vi "Add Configuration Controls.vi"(0 "New Code Module":path, 1 "vi reference":refnum<vi>, 2 "Configuration Ctl Refnum":refnum<vi>, 11 "error in (no error)":errorcluster) -> (4 "Controls Reference":refnum<vi>[](array[refnum]), 15 "error out":errorcluster)   [LabVIEW 2021, in "Migrator.lvlib"]
uses:
  Migrator.lvlib
  Migrator Reusables/Migrator Reusables.lvlib
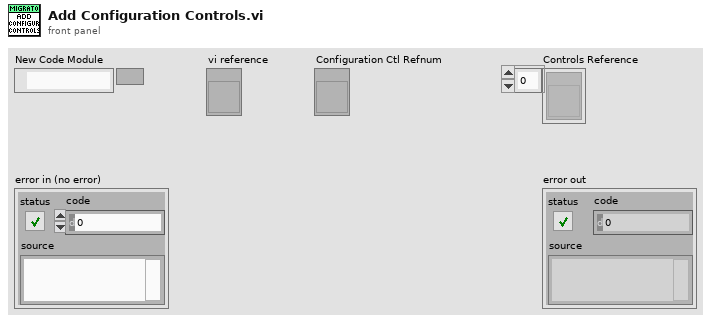
[diagram p1: front panel]
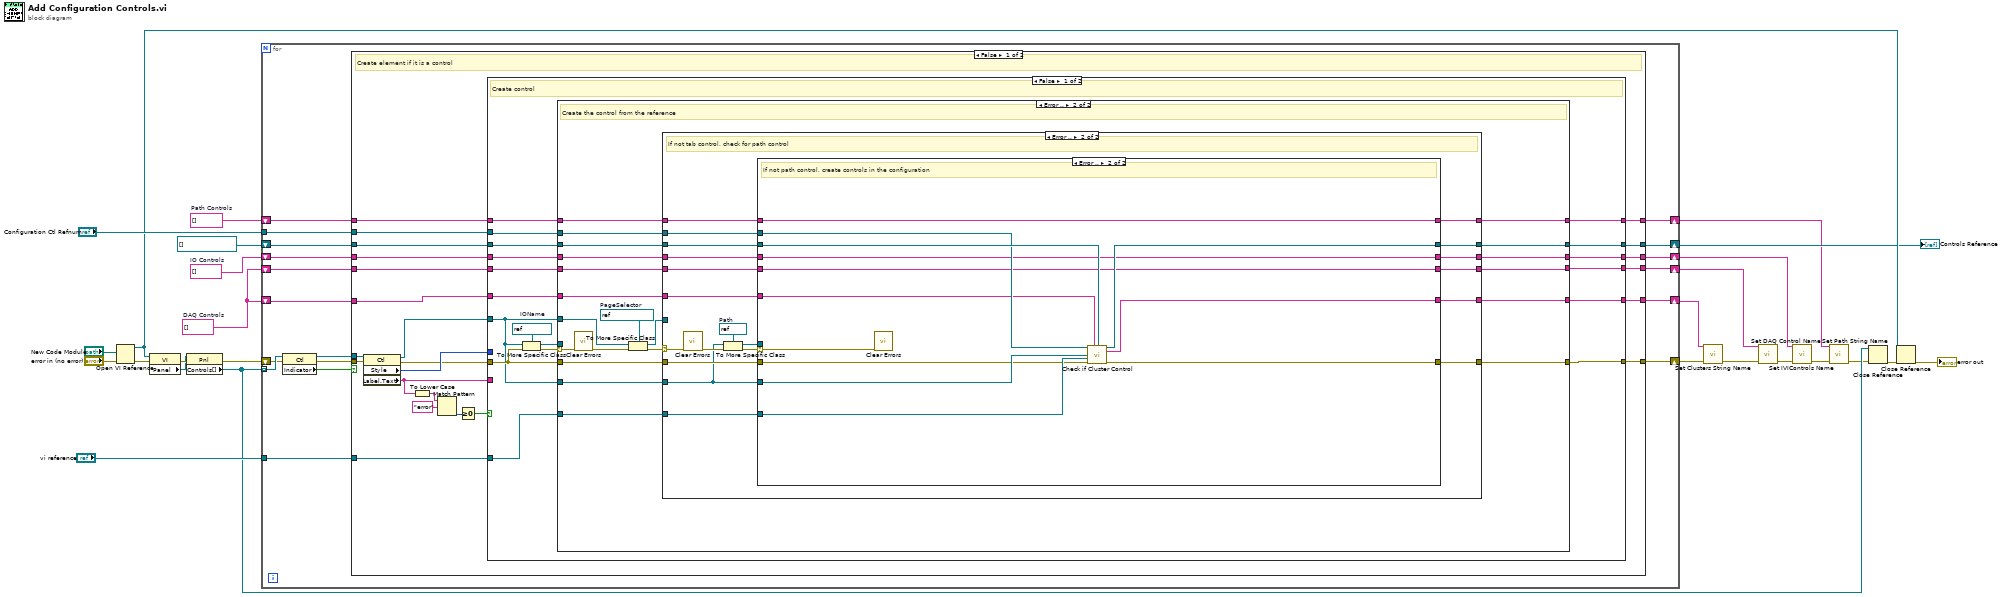
[diagram p0: block diagram]
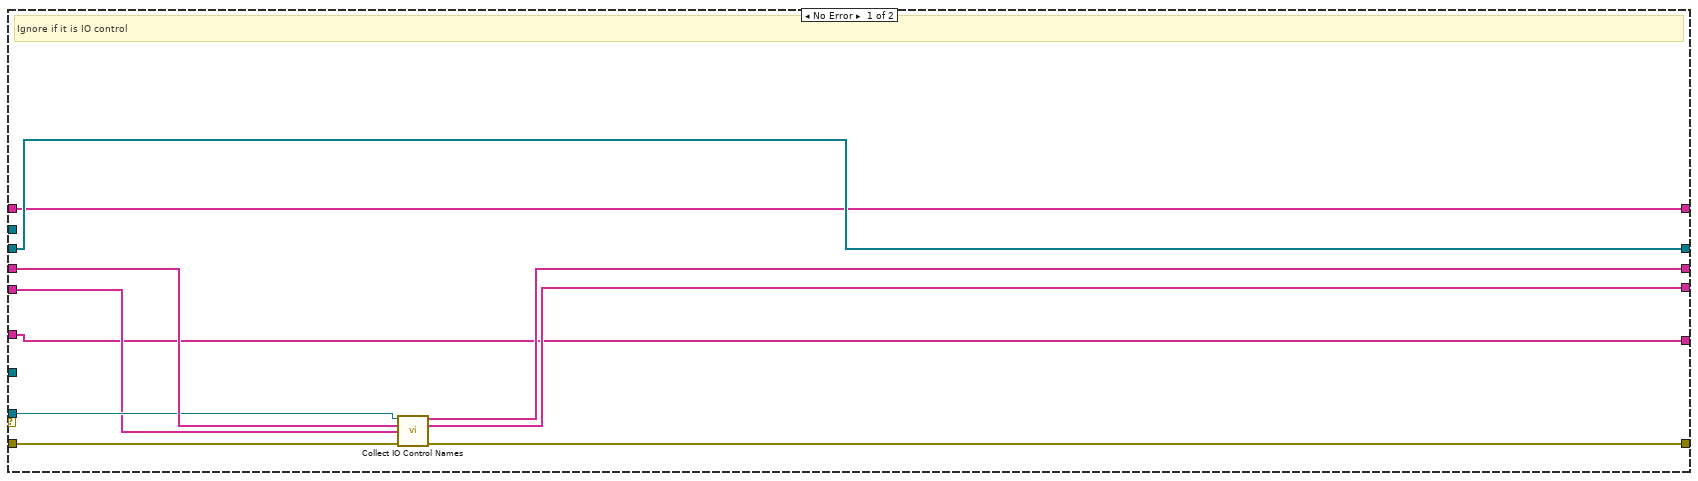
[diagram p2: hidden frame]
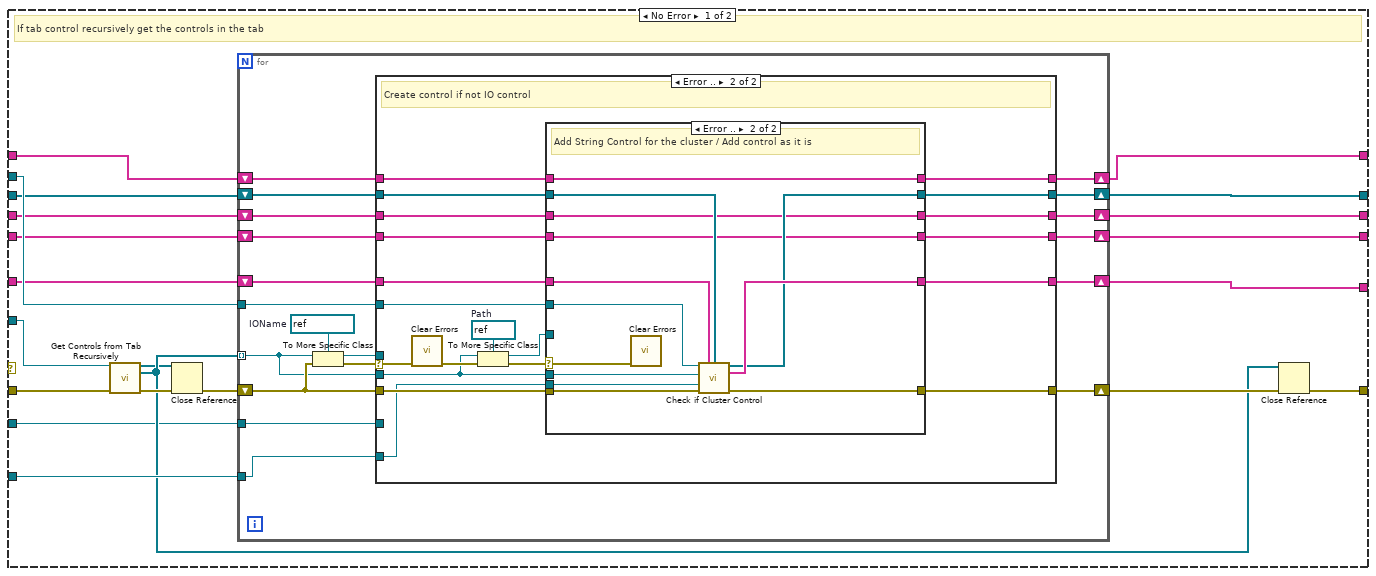
[diagram p3: hidden frame]
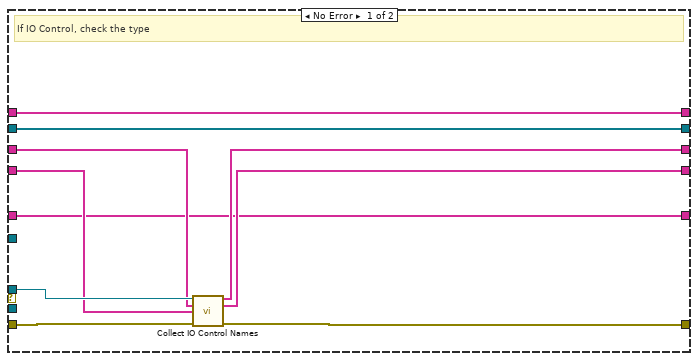
[diagram p4: hidden frame]
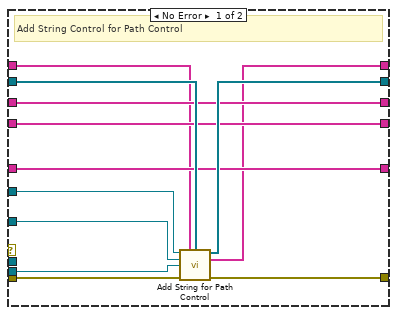
[diagram p5: hidden frame]
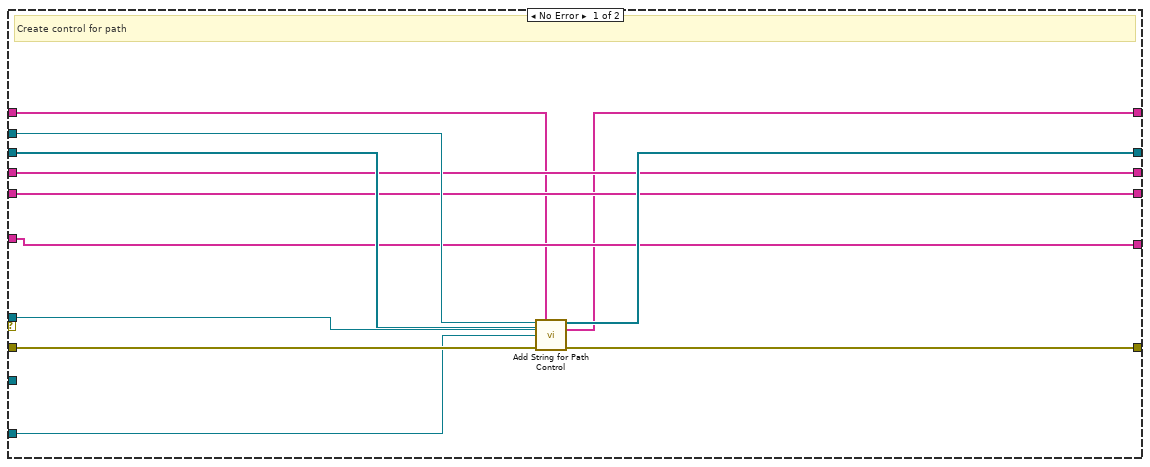
[diagram p6: hidden frame]
diagram:
  w4 = string[] []  # Path Controls
  w8 = string[] []  # DAQ Controls
  w12 = string[] []  # IO Controls
  n1 = Open VI Reference(vi path="New Code Module", error in (no error)="error in (no error)") -> (vi reference=w18:refnum<vi>, error out=w16:errorcluster)  [unwired: 4 in]
  n2 = property class="VI"(reference=w18, error in=w16) -> (error out=w20:errorcluster, "Panel"=w19:refnum<vi>)  [unwired: 1 out]
  n3 = property class="Pnl"(reference=w19, error in=w20) -> (error out=w15:errorcluster, "Controls[]"=w17:refnum<vi>[])  [unwired: 1 out]
  n4 = for {
    tunnel: w17 -> [w42] mode=indexing
    shift-right: [w43] -> w5
    shift-left: w15 -> [w40]
    tunnel: "Configuration Ctl Refnum" -> [w44]
    tunnel: "vi reference" -> [w37]
    shift-right: [w36] -> w14
    shift-left: refnum<vi>[] [] -> [w35]
    shift-right: [w33] -> w13
    shift-left: w12 -> [w34]
    shift-right: [w31] -> w10
    shift-left: w8 -> [w32]
    shift-right: [w30] -> w7
    shift-left: w8 -> [w29]
    shift-right: [w27] -> w3
    shift-left: w4 -> [w28]
    n5 = property class="Ctl"(reference=w42, error in=w40) -> (reference out=w38:refnum<vi>, error out=w39:errorcluster, "Indicator"=w41:bool)
    n6 = case shown="False" w41 {
      tunnel: w44 -> [w66 _]
      tunnel: w39 -> [w65 w268]
      tunnel: w38 -> [w63 _]
      tunnel: [w62 w268] -> w43
      tunnel: w37 -> [w55 _]
      tunnel: [w54 w267] -> w36
      tunnel: w35 -> [w53 w267]
      tunnel: w34 -> [w52 w266]
      tunnel: [w51 w266] -> w33
      tunnel: w32 -> [w50 w265]
      tunnel: [w49 w265] -> w31
      tunnel: [w48 w264] -> w30
      tunnel: w29 -> [w47 w264]
      tunnel: w28 -> [w46 w263]
      tunnel: [w45 w263] -> w27
      frame False {
        # "Create element if it is a control"
        n7 = property class="Ctl"(reference=w63, error in=w65) -> (reference out=w56:refnum<vi>, error out=w64:errorcluster, "Style"=w67:u32, "Label.Text"=w61:string)
        n8 = To Lower Case(string=w61) -> (all lower case string=w57:string)
        n9 = Match Pattern(string=w57, regular expression="error") -> (offset past match=w59:i32)  [unwired: 1 in, 3 out]
        n10 = Greater Or Equal To 0?(x=w59) -> (x >= 0?=w58:bool)
        n11 = case shown="False" w58 {
          tunnel: w67 -> [_ _]
          tunnel: w66 -> [w83 _]
          tunnel: w64 -> [w85 w262]
          tunnel: w56 -> [w78 _]
          tunnel: w61 -> [_ _]
          tunnel: [w84 w262] -> w62
          tunnel: w55 -> [w82 _]
          tunnel: [w77 w261] -> w54
          tunnel: w53 -> [w76 w261]
          tunnel: w52 -> [w75 w260]
          tunnel: [w74 w260] -> w51
          tunnel: w50 -> [w73 w259]
          tunnel: [w72 w259] -> w49
          tunnel: [w71 w258] -> w48
          tunnel: w47 -> [w70 w258]
          tunnel: w46 -> [w69 w257]
          tunnel: [w68 w257] -> w45
          frame False {
            w81 = refnum<vi> refnum  # IOName
            # "Create control"
            n12 = To More Specific Class(target class=w81, reference=w78, error in=w85) -> (specific class reference=w79:refnum<vi>, error out=w80:errorcluster)
            n13 = case shown="Error .." w80 {
              selector: w80 -> [_ w113]
              tunnel: w82 -> [_ w110]
              tunnel: w78 -> [_ w116]
              tunnel: w83 -> [_ w115]
              tunnel: [w95 w114] -> w84
              tunnel: w85 -> [w91 w112]
              tunnel: w79 -> [w90 _]
              tunnel: w78 -> [_ w108]
              tunnel: [w94 w105] -> w77
              tunnel: w76 -> [w94 w104]
              tunnel: w75 -> [w93 w103]
              tunnel: [w92 w102] -> w74
              tunnel: w73 -> [w89 w101]
              tunnel: [w88 w100] -> w72
              tunnel: [w87 w99] -> w71
              tunnel: w70 -> [w87 w98]
              tunnel: w69 -> [w86 w97]
              tunnel: [w86 w96] -> w68
              frame No Error {
                # "Ignore if it is IO control"
                n14 = call "Collect IO Control Names.vi"("IO Control"=w90, "IO Controls in"=w93, "DAQ Controls in"=w89, "error in (no error)"=w91) -> ("IO Controls out"=w92:string[], "DAQ Controls out"=w88:string[], "error out"=w95:errorcluster)  [unwired: 9 in]
              }
              frame Error {
                w111 = refnum<vi> refnum  # PageSelector
                # "Create the control from the reference"
                n15 = call <vilib>:"Clear Errors.vi"("error in (no error)"=w113) -> ("error out"=w109:errorcluster)  [unwired: 5 in, 1 out]
                n16 = To More Specific Class(target class=w111, reference=w108, error in=w109) -> (specific class reference=w106:refnum<vi>, error out=w107:errorcluster)
                n17 = case shown="Error .." w107 {
                  selector: w107 -> [_ w223]
                  tunnel: w110 -> [w134 w229]
                  tunnel: w116 -> [w123 w214]
                  tunnel: w115 -> [w133 w227]
                  tunnel: [w137 w228] -> w114
                  tunnel: w112 -> [w136 w224]
                  tunnel: w106 -> [w135 _]
                  tunnel: [w121 w230] -> w105
                  tunnel: w104 -> [w122 w231]
                  tunnel: w103 -> [w132 w219]
                  tunnel: [w131 w216] -> w102
                  tunnel: w101 -> [w125 w218]
                  tunnel: [w124 w215] -> w100
                  tunnel: [w119 w226] -> w99
                  tunnel: w98 -> [w120 w225]
                  tunnel: w97 -> [w118 w213]
                  tunnel: [w117 w212] -> w96
                  frame No Error {
                    # "If tab control recursively get the controls in the tab"
                    n18 = call "Get Controls from Tab Recursively.vi"("PageSel Refnum"=w135, "error in (no error)"=w136) -> ("Indicators in Tab"=w126:refnum<vi>[], "Controls in Tab"=w127:refnum<vi>[], "error out"=w129:errorcluster)  [unwired: 11 in]
                    n19 = Close Reference(reference=w126, error in (no error)=w129) -> (error out=w128:errorcluster)
                    n20 = for {
                      tunnel: w127 -> [w142] mode=indexing
                      tunnel: w134 -> [w145]
                      tunnel: w133 -> [w147]
                      shift-right: [w150] -> w131
                      shift-left: w132 -> [w154]
                      shift-right: [w151] -> w130
                      shift-left: w128 -> [w148]
                      shift-right: [w149] -> w124
                      shift-left: w125 -> [w152]
                      tunnel: w123 -> [w146]
                      shift-right: [w143] -> w121
                      shift-left: w122 -> [w144]
                      shift-right: [w140] -> w119
                      shift-left: w120 -> [w141]
                      shift-right: [w138] -> w117
                      shift-left: w118 -> [w139]
                      w156 = refnum<vi> refnum  # IOName
                      n21 = To More Specific Class(target class=w156, reference=w142, error in=w148) -> (specific class reference=w155:refnum<vi>, error out=w153:errorcluster)
                      n22 = case shown="Error .." w153 {
                        selector: w153 -> [_ w176]
                        tunnel: w155 -> [w166 _]
                        tunnel: w154 -> [w165 w172]
                        tunnel: w152 -> [w164 w170]
                        tunnel: [w163 w182] -> w151
                        tunnel: [w162 w171] -> w150
                        tunnel: [w161 w169] -> w149
                        tunnel: w148 -> [w160 w183]
                        tunnel: w147 -> [_ w184]
                        tunnel: w146 -> [_ _]
                        tunnel: w145 -> [_ w181]
                        tunnel: [w159 w179] -> w143
                        tunnel: w144 -> [w159 w180]
                        tunnel: w142 -> [_ w174]
                        tunnel: w141 -> [w158 w186]
                        tunnel: [w158 w185] -> w140
                        tunnel: w139 -> [w157 w168]
                        tunnel: [w157 w167] -> w138
                        frame No Error {
                          # "If IO Control, check the type"
                          n23 = call "Collect IO Control Names.vi"("IO Control"=w166, "IO Controls in"=w165, "DAQ Controls in"=w164, "error in (no error)"=w160) -> ("IO Controls out"=w162:string[], "DAQ Controls out"=w161:string[], "error out"=w163:errorcluster)  [unwired: 9 in]
                        }
                        frame Error {
                          w178 = refnum<vi> refnum  # Path
                          # "Create control if not IO control"
                          n24 = call <vilib>:"Clear Errors.vi"("error in (no error)"=w176) -> ("error out"=w175:errorcluster)  [unwired: 5 in, 1 out]
                          n25 = To More Specific Class(target class=w178, reference=w174, error in=w175) -> (specific class reference=w173:refnum<vi>, error out=w177:errorcluster)
                          n26 = case shown="Error .." w177 {
                            selector: w177 -> [_ w211]
                            tunnel: w186 -> [w189 w210]
                            tunnel: [w189 w209] -> w185
                            tunnel: w184 -> [w195 w208]
                            tunnel: w183 -> [w198 w207]
                            tunnel: [w197 w206] -> w182
                            tunnel: w174 -> [_ w205]
                            tunnel: w181 -> [w194 w204]
                            tunnel: w180 -> [w193 w203]
                            tunnel: [w192 w202] -> w179
                            tunnel: w173 -> [w196 _]
                            tunnel: [w191 w201] -> w171
                            tunnel: w172 -> [w191 w201]
                            tunnel: w170 -> [w190 w200]
                            tunnel: [w190 w200] -> w169
                            tunnel: w168 -> [w188 w199]
                            tunnel: [w187 w199] -> w167
                            frame No Error {
                              # "Add String Control for Path Control"
                              n27 = call "Add String for Path Control.vi"("String Controls in"=w195, "String Names in"=w188, "Controls Ref IN"=w193, "Path Refnum"=w196, "vi reference"=w194, "error in (no error)"=w198) -> ("Controls Ref Out"=w192:refnum<vi>[], "String Names Out"=w187:string[], "error out"=w197:errorcluster)  [unwired: 7 in]
                            }
                            frame Error {
                              # "Add String Control for the cluster / Add control as it is"
                              n28 = call <vilib>:"Clear Errors.vi"("error in (no error)"=w211) -> ()  [unwired: 5 in, 2 out]
                              n29 = call "Check if Cluster Control.vi"(0:"String Controls in"=w208, 1:"String Controls in"=w210, "Controls Ref IN"=w203, "Ctl Refnum"=w205, "vi reference"=w204, "error in"=w207) -> ("Controls Ref Out"=w202:refnum<vi>[], "String Controls out"=w209:string[], "error out"=w206:errorcluster)  [unwired: 7 in]
                            }
                          }
                        }
                      }
                    }
                    n30 = Close Reference(reference=w127, error in (no error)=w130) -> (error out=w137:errorcluster)
                  }
                  frame Error {
                    w220 = refnum<vi> refnum  # Path
                    # "If not tab control, check for path control"
                    n31 = call <vilib>:"Clear Errors.vi"("error in (no error)"=w223) -> ("error out"=w222:errorcluster)  [unwired: 5 in, 1 out]
                    n32 = To More Specific Class(target class=w220, reference=w214, error in=w222) -> (specific class reference=w217:refnum<vi>, error out=w221:errorcluster)
                    n33 = case shown="Error .." w221 {
                      selector: w221 -> [_ w247]
                      tunnel: w231 -> [w239 w256]
                      tunnel: [w237 w255] -> w230
                      tunnel: w229 -> [w242 w254]
                      tunnel: [w238 w253] -> w228
                      tunnel: w227 -> [w240 w252]
                      tunnel: w214 -> [_ w251]
                      tunnel: [w234 w250] -> w226
                      tunnel: w225 -> [w234 w249]
                      tunnel: w224 -> [w243 w248]
                      tunnel: w219 -> [w236 w246]
                      tunnel: w218 -> [w235 w245]
                      tunnel: w217 -> [w241 _]
                      tunnel: [w236 w246] -> w216
                      tunnel: [w235 w245] -> w215
                      tunnel: w213 -> [w233 w244]
                      tunnel: [w232 w244] -> w212
                      frame No Error {
                        # "Create control for path"
                        n34 = call "Add String for Path Control.vi"("String Controls in"=w240, "String Names in"=w233, "Controls Ref IN"=w239, "Path Refnum"=w241, "vi reference"=w242, "error in (no error)"=w243) -> ("Controls Ref Out"=w237:refnum<vi>[], "String Names Out"=w232:string[], "error out"=w238:errorcluster)  [unwired: 7 in]
                      }
                      frame Error {
                        # "If not path control, create controls in the configuration"
                        n35 = call <vilib>:"Clear Errors.vi"("error in (no error)"=w247) -> ()  [unwired: 5 in, 2 out]
                        n36 = call "Check if Cluster Control.vi"(0:"String Controls in"=w252, 1:"String Controls in"=w249, "Controls Ref IN"=w256, "Ctl Refnum"=w251, "vi reference"=w254, "error in"=w248) -> ("Controls Ref Out"=w255:refnum<vi>[], "String Controls out"=w250:string[], "error out"=w253:errorcluster)  [unwired: 7 in]
                      }
                    }
                  }
                }
              }
            }
          }
          frame True {
            # "Ignore if it is error control"
          }
        }
      }
      frame True {
        # "Ignore if it is indicator"
      }
    }
  }
  "Controls Reference" <- w14
  n37 = call "Set Clusters String Name.vi"("Conmtrols Name"=w7, "error in (no error)"=w5) -> ("error out"=w6:errorcluster)  [unwired: 13 in]
  n38 = call "Set DAQ Control Name.vi"("Conmtrols Name"=w10, "error in (no error)"=w6) -> ("error out"=w9:errorcluster)  [unwired: 13 in]
  n39 = call "Set IVIControls Name.vi"("Conmtrols Name"=w13, "error in (no error)"=w9) -> ("error out"=w2:errorcluster)  [unwired: 13 in]
  n40 = call "Set Path String Name.vi"("Controls Name"=w3, "error in (no error)"=w2) -> ("error out"=w1:errorcluster)  [unwired: 13 in]
  n41 = Close Reference(reference=w17, error in (no error)=w1) -> (error out=w23:errorcluster)
  n42 = Close Reference(reference=w18, error in (no error)=w23) -> (error out=→"error out":errorcluster)
